vi "All Tests.vi"(8 "error in (no error)":errorcluster) -> (0 "error out":errorcluster)   [LabVIEW 2020]
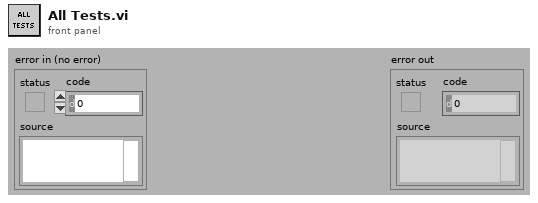
[diagram p1: front panel]
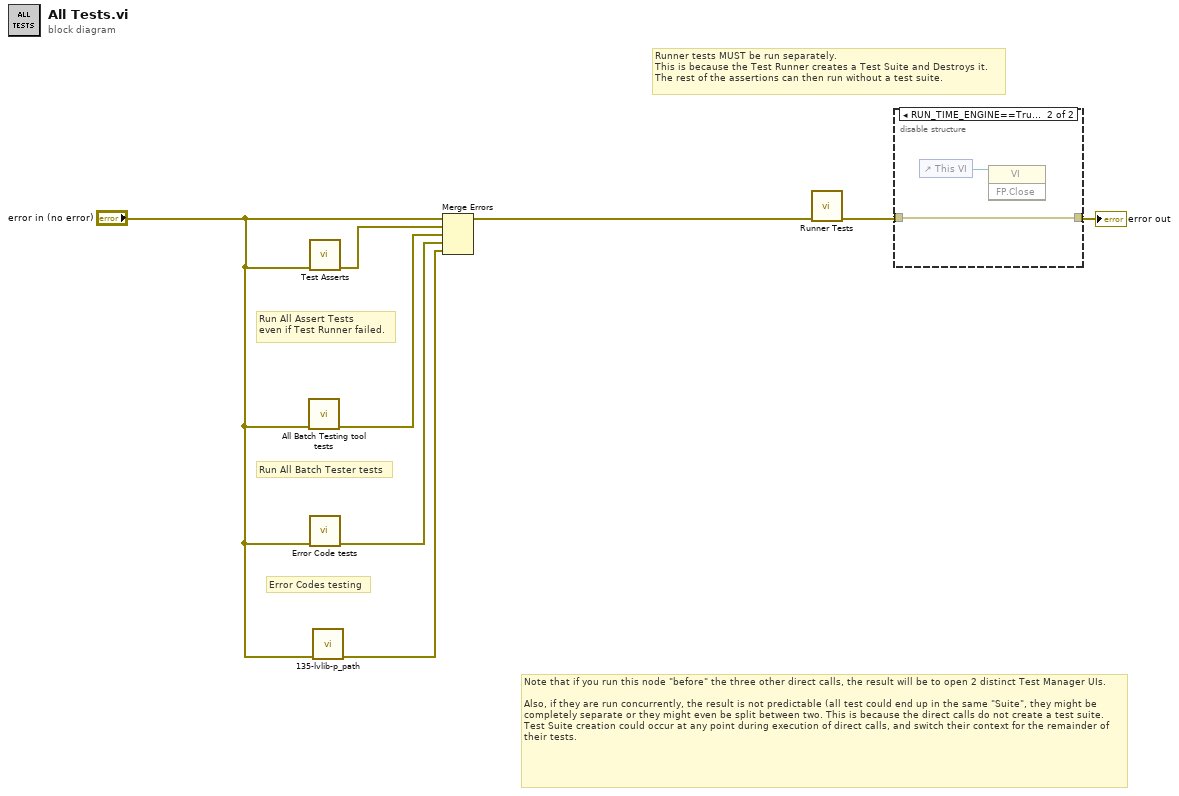
[diagram p0: block diagram]
diagram:
  # "Error Codes testing"
  # "Run All Batch Tester tests"
  # "Run All Assert Tests\neven if Test Runner failed."
  # "Note that if you run this node \"before\" the three other direct calls, the result will be to open 2 distinct Test Manager UIs.\n\nAlso, if they are run concurrently, the result is not predictable (all test could end up in the same \"Suite\", they might be completely separate or they might even be split between two. This is because the direct calls do not create a test suite. Test Suite creation could occur at any point during execution of direct calls, and switch their context for the remainder of their tests."
  # "Runner tests MUST be run separately.\nThis is because the Test Runner creates a Test Suite and Destroys it.\nThe rest of the assertions can then run without a test suite."
  n1 = call "All Batch Testing tool tests.vi"("error in (no error)"="error in (no error)") -> ("error out"=w3:errorcluster)  [unwired: 10 in]
  n2 = call "Test Asserts.vi"("error in (no error)"="error in (no error)") -> ("error out"=w4:errorcluster)  [unwired: 10 in]
  n3 = call "Error Code tests.vi"("error in (no error)"="error in (no error)") -> ("error out"=w2:errorcluster)  [unwired: 10 in]
  n4 = call "135-lvlib-p_path.vi"("error in (no error)"="error in (no error)") -> ("error out"=w1:errorcluster)  [unwired: 10 in]
  n5 = Merge Errors("error in (no error)", w4, w3, w2, w1) -> (w6:errorcluster)
  n6 = call "Runner Tests.vi"("error in (no error)"=w6) -> ("error out"=w7:errorcluster)  [unwired: 10 in]
  n7 = disable-structure shown="RUN_TIME_ENGINE==True" {
    disable-tunnel: w7 -> [w9 w10]
    disable-tunnel: [w9 w10] -> w8
    frame condition #0 (active) {
    }
    frame condition #1 {
      n8 = control-ref of="This VI"() -> (w11:refnum<vi>)
      n9 = invoke class="VI" method="FP.Close"(reference=w11) -> ()  [unwired: 2 in, 3 out]
    }
  }
  "error out" <- w8
